vi "EnumerateElements.vi"(8 "error in (no error)":errorcluster, 10 "Qualified Name":string, 11 "ConfigManager.Text in":refnum<class "ConfigManager.Text.lvclass">) -> (0 "error out":errorcluster, 2 "keys":string[](array[string]), 3 "ConfigManager.Text out":refnum<class "ConfigManager.Text.lvclass">)   [LabVIEW 2013, in "CfgManager.Text.lvlib" / "ConfigManager.Text.lvclass"]
uses:
  ConfigManager.Text.lvclass
  ConfigManager.Text.lvclass/ConfigManager.Text.ctl
  <vilib>/LabVIEW Open Source Project/Unicity/Delimiter/Delimiter.lvclass
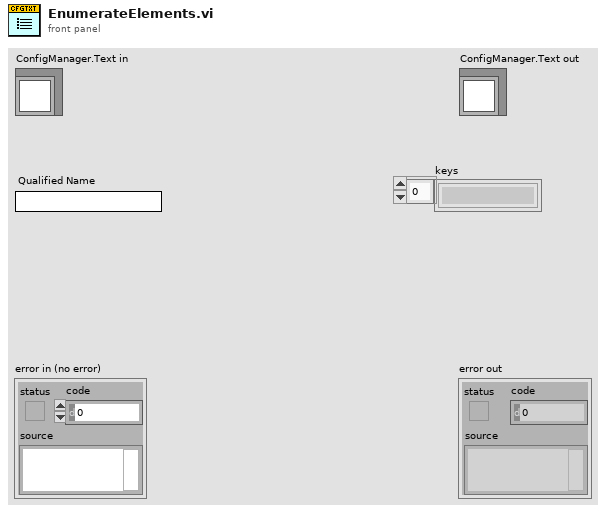
[diagram p1: front panel]
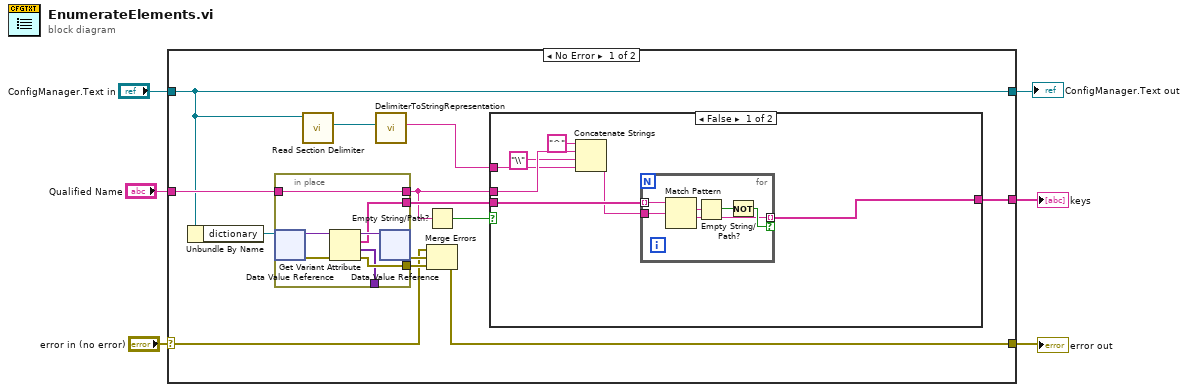
[diagram p0: block diagram]
diagram:
  n1 = case shown="No Error" "error in (no error)" {
    selector: "error in (no error)" -> [w15 w42]
    tunnel: [w19 w42] -> w1
    tunnel: "ConfigManager.Text in" -> [w8 w41]
    tunnel: [w8 w41] -> w5
    tunnel: [w10 _] -> w3
    tunnel: "Qualified Name" -> [w14 _]
    frame No Error {
      n2 = Unbundle By Name(w8) -> ("dictionary"=w16:refnum<data-value>)
      n3 = in-place {
        in-place-border: [w35] -> w18
        in-place-border: w14 -> [w36]
        in-place-border: [w37] -> w13
        in-place-border: [w36] -> w12
        in-place-border: [w34] -> _
        n4 = in-place-dvr #1(w16) -> (w39:variant, w40:errorcluster)
        n5 = Get Variant Attribute(Variant=w39, error in=w40) -> (duplicate Variant=w38:variant, names=w37:string[], values=w34:variant[], error out=w35:errorcluster)  [unwired: 2 in]
        n6 = in-place-dvr #1(w38) -> (w17:errorcluster)  [unwired: 1 out]
      }
      n7 = call "Read Section Delimiter.vi"("ConfigManager.Text in"=w8) -> ("Section Delimiter"=w7:refnum<class "Delimiter.lvclass">)  [unwired: 9 in, 1 out]
      n8 = call <vilib>:"DelimiterToStringRepresentation.vi"("Delimiter"=w7) -> ("String representation"=w9:string)  [unwired: 10 in]
      n9 = Empty String/Path?(string/path=w12) -> (empty?=w11:bool)
      n10 = Merge Errors(w15, w17, w18) -> (w19:errorcluster)
      n11 = case shown="False" w11 {
        tunnel: w13 -> [w26 w33]
        tunnel: w12 -> [w25 _]
        tunnel: [w20 w33] -> w10
        tunnel: w9 -> [w22 _]
        frame False {
          n12 = Concatenate Strings("^" ("string"), w25, "\\" ("string"), w22) -> (w24:string)
          n13 = for {
            tunnel: w24 -> [w29]
            tunnel: w26 -> [w30] mode=indexing
            tunnel: [w27] -> w20 mode=indexing if=w28
            n14 = Match Pattern(string=w30, regular expression=w29) -> (match substring=w32:string, after substring=w27:string)  [unwired: 1 in, 2 out]
            n15 = Empty String/Path?(string/path=w32) -> (empty?=w31:bool)
            n16 = Not(x=w31) -> (.not. x?=w28:bool)
          }
        }
        frame True {
        }
      }
    }
    frame Error {
    }
  }
  "error out" <- w1
  "ConfigManager.Text out" <- w5
  "keys" <- w3
